vi "Popup alerte régulateurs.vi"(2 "Message":string, 3 "Problème":string) -> ()   [LabVIEW 2022 SP3]
panel:
  in  "BtnOn":bool
  # "alerte régulateur"
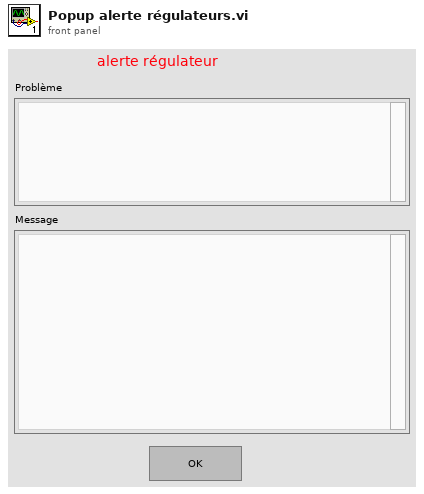
[diagram p1: front panel]
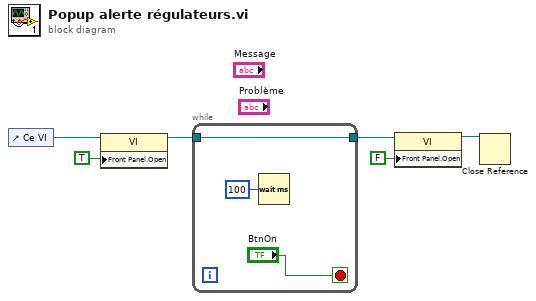
[diagram p0: block diagram]
diagram:
  n1 = control-ref of="Ce VI"() -> (w6:refnum<vi>)
  n2 = property class="VI"(reference=w6, "Front Panel.Open"=TRUE ("Fenêtre face-avant:Ouverte")) -> (reference out=w5:refnum<vi>)  [unwired: 1 in, 1 out]
  n3 = while {
    tunnel: w5 -> [w7]
    tunnel: [w7] -> w4
    stop <- "BtnOn" stop-if-true
    n4 = Wait (ms)(milliseconds to wait=u32 100 ("attente (ms)")) -> ()  [unwired: 1 out]
  }
  n5 = property class="VI"(reference=w4, "Front Panel.Open"=FALSE ("Fenêtre face-avant:Ouverte")) -> (reference out=w3:refnum<vi>)  [unwired: 1 in, 1 out]
  n6 = Close Reference(reference=w3) -> ()  [unwired: 1 in, 1 out]
